vi "Compare Versions.vi"(10 "Version 2":string, 11 "Version 1":string) -> (1 "Version 1 Lesser?":bool, 2 "Equal?":bool, 3 "Version 1 Greater?":bool)   [LabVIEW 2016, in "SLL Application.lvlib"]
doc: "Compares two versions and returns whether the version 1 is greater, or equal to, or lesser than what is specified for version 2.\n\nThe number of digits in the version number can also vary which is also handled. Eg:\nVersion 1: 1.0.\nVersion 2: 1.0.0.1"
uses:
  SLL Application.lvlib
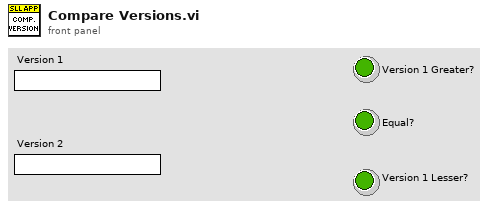
[diagram p1: front panel]
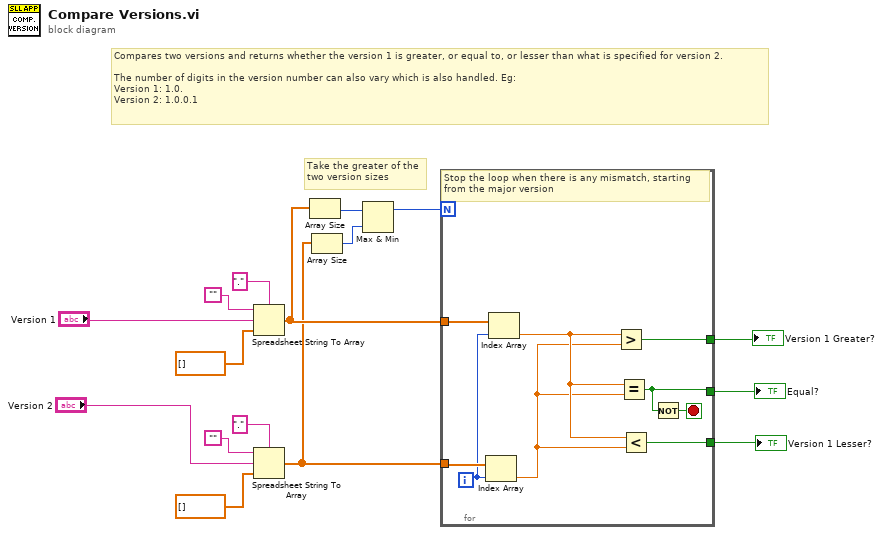
[diagram p0: block diagram]
diagram:
  # "Compares two versions and returns whether the version 1 is greater, or equal to, or lesser than what is specified for version 2.\n\nThe number of digits in the version number can also vary which is also handled. Eg:\nVersion 1: 1.0.\nVersion 2: 1.0.0.1"
  # "Take the greater of the\ntwo version sizes"
  n1 = Spreadsheet String To Array(delimiter (Tab)=".", format string="", spreadsheet string="Version 1", array type (2D Dbl)=dbl[] []) -> (array=w5:dbl[])
  n2 = Spreadsheet String To Array(delimiter (Tab)=".", format string="", spreadsheet string="Version 2", array type (2D Dbl)=dbl[] []) -> (array=w4:dbl[])
  n3 = Array Size(array=w5) -> (size(s)=w8:i32)
  n4 = Array Size(array=w4) -> (size(s)=w7:i32)
  n5 = Max & Min(x=w8, y=w7) -> (max(x,y)=w6:i32)  [unwired: 1 out]
  n6 = for {
    N: w6 -> [_]
    tunnel: w5 -> [w25]
    tunnel: w4 -> [w24]
    tunnel: [w19] -> w3
    tunnel: [w18] -> w1
    tunnel: [w17] -> w2
    i -> [w23]
    stop <- w20 stop-if-true
    # "Stop the loop when there is any mismatch, starting from the major version"
    n7 = Index Array(array=w24, index=w23) -> (element=w21:dbl)
    n8 = Index Array(array=w25, index=w23) -> (element=w22:dbl)
    n9 = Greater?(x=w22, y=w21) -> (0:w19:bool)
    n10 = Equal?(x=w22, y=w21) -> (x = y?=w17:bool)
    n11 = Less?(x=w22, y=w21) -> (x < y?=w18:bool)
    n12 = Not(x=w17) -> (.not. x?=w20:bool)
  }
  "Version 1 Greater?" <- w3
  "Equal?" <- w2
  "Version 1 Lesser?" <- w1
